vi "OverlayLabeledRectangle.vi"   [LabVIEW 2020, in "OpenLvVision_Overlays.lvlib"]
doc: "Overlays an rectangle with text on top of an image."
uses:
  OpenLvVision_Overlays.lvlib
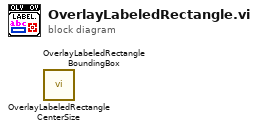
[diagram p0: block diagram]
diagram:
  n1 = call "OverlayLabeledRectangleCenterSize.vi"() -> ()  [unwired: 10 in, 2 out]
  n2 = call "OverlayLabeledRectangleBoundingBox.vi"() -> ()  [unwired: 10 in, 2 out]
